vi "Get Pressed Button Index.vi"(8 "error in":errorcluster, 11 "Buttons":T1) -> (0 "error out":errorcluster, 3 "Button Index":i32)   [LabVIEW 2026]
doc: "Takes one of the ATM front-panel function button clusters (Left Buttons or Right Buttons) and returns the index of the button that is TRUE: 0 for the top button, 1 for the middle, 2 for the bottom. Returns -1 when no button is TRUE. If several are TRUE the topmost one wins.\n\nError behaviour: error in is passed to error out unchanged; the index is computed in every case."
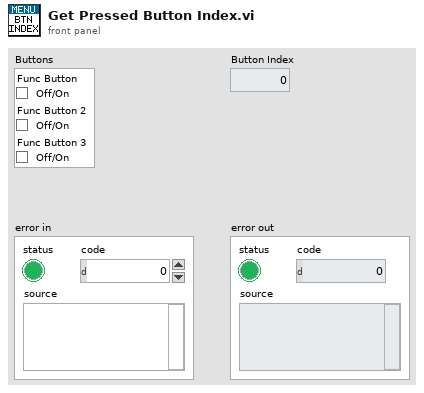
[diagram p1: front panel]
types:
  T1 = cluster{"Func Button":bool, "Func Button 2":bool, "Func Button 3":bool}
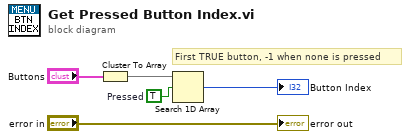
[diagram p0: block diagram]
diagram:
  w3 = TRUE  # Pressed
  # "First TRUE button, -1 when none is pressed"
  n1 = Cluster To Array(cluster="Buttons") -> (array=w4:bool[])
  n2 = Search 1D Array(1D array=w4, element=w3) -> (index of element=→"Button Index":i32)  [unwired: 1 in]
  "error out" <- "error in"
